vi "Radio Read.vi"() -> ()   [LabVIEW 2013]
uses:
  <vilib>/Instr/_visa.llb/VISA Configure Serial Port (Instr).vi
panel:
  out "Z":dbl(slide) scale=-90.0..90.0
  out "Y":dbl(slide) scale=-90.0..90.0
  out "X":dbl(slide) scale=-90.0..90.0
  out "ELEV":dbl(slide) scale=1000.0..2000.0
  out "ALE":dbl(slide) scale=1000.0..2000.0
  out "THRO":dbl(slide) scale=1000.0..2000.0
  out "RUDD":dbl(slide) scale=1000.0..2000.0
  in  "Stop Button":bool
  out "read buffer":string
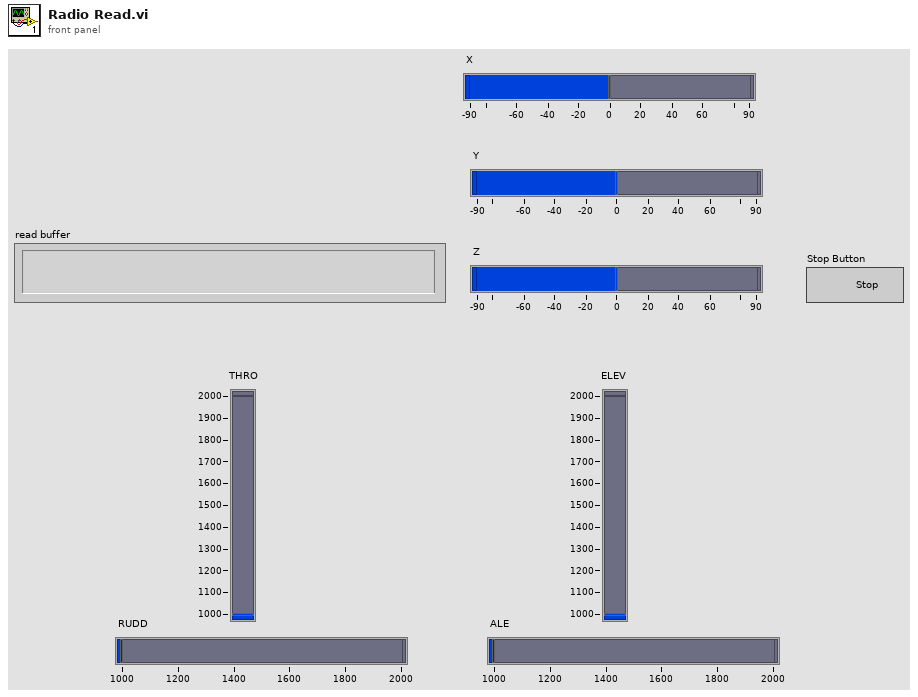
[diagram p1: front panel]
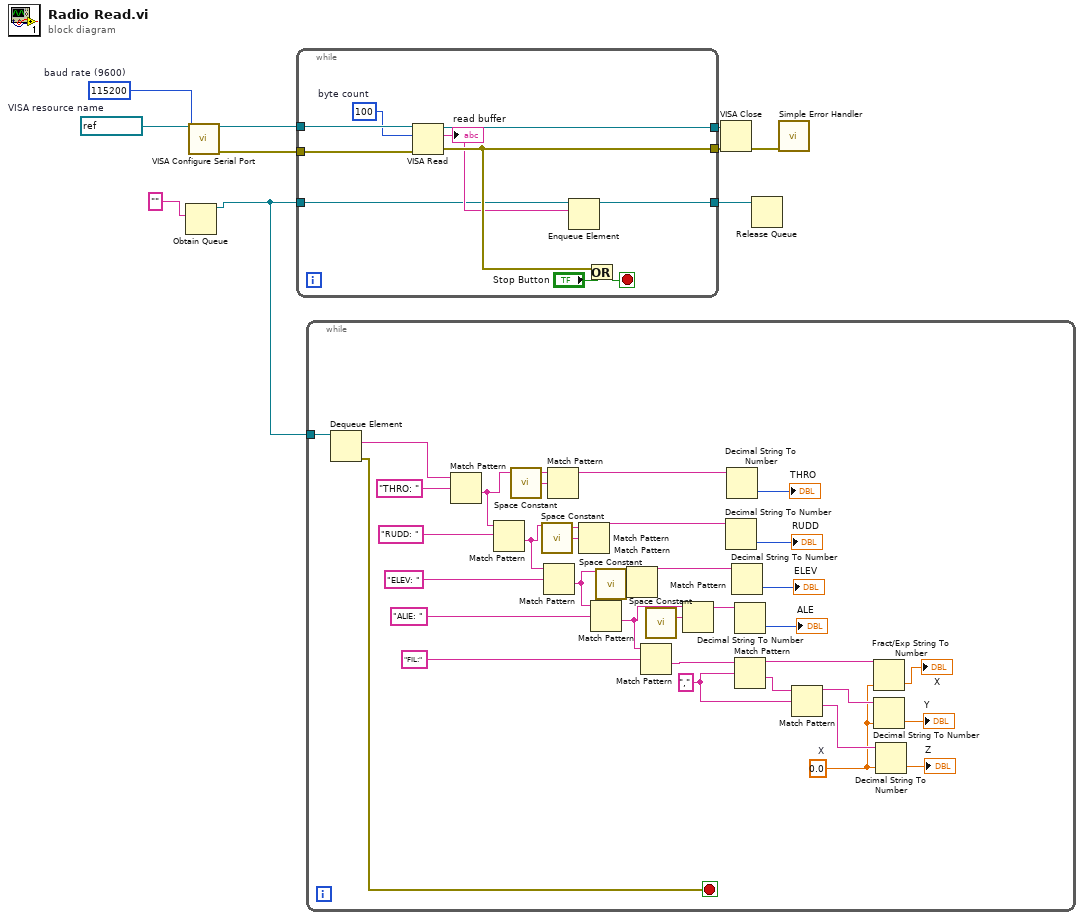
[diagram p0: block diagram]
diagram:
  w1 = u32 115200  # baud rate (9600)
  w8 = refnum<visa-resource-name> "COM3"  # VISA resource name
  n1 = Obtain Queue(element data type="") -> (queue out=w3:refnum<queue>)  [unwired: 4 in, 2 out]
  n2 = call-poly "VISA Configure Serial Port"("VISA resource name"=w8, "baud rate (9600)"=w1) -> ("VISA resource name out"=w6:refnum<visa-resource-name>, "error out"=w7:errorcluster)  [unwired: 12 in]
  n3 = while {
    tunnel: [w20] -> w10
    tunnel: [w18] -> w9
    tunnel: w7 -> [w19]
    tunnel: w6 -> [w15]
    tunnel: w3 -> [w12]
    tunnel: [w11] -> w2
    stop <- w16 stop-if-true
    w14 = u32 100  # byte count
    n4 = VISA Read(VISA resource name=w15, byte count=w14, error in (no error)=w19) -> (VISA resource name out=w20:refnum<visa-resource-name>, read buffer=w13:string, error out=w18:errorcluster)  [unwired: 1 out]
    "read buffer" <- w13
    n5 = Enqueue Element(queue=w12, element=w13) -> (queue out=w11:refnum<queue>)  [unwired: 2 in, 2 out]
    n6 = Or(x=w18, y="Stop Button") -> (x .or. y?=w16:bool)
  }
  n7 = while {
    tunnel: w3 -> [w54]
    stop <- w48 stop-if-true
    w22 = 0.0  # X
    w28 = "," ("regular expression")
    n8 = Dequeue Element(queue=w54) -> (element=w52:string, error out=w48:errorcluster)  [unwired: 2 in, 2 out]
    n9 = Match Pattern(string=w52, regular expression="THRO: ") -> (after substring=w49:string)  [unwired: 1 in, 3 out]
    n10 = Match Pattern(string=w49, regular expression="RUDD: ") -> (after substring=w44:string)  [unwired: 1 in, 3 out]
    n11 = call <vilib>:"Space Constant.vi"() -> ("String"=w51:string)
    n12 = call <vilib>:"Space Constant.vi"() -> ("String"=w50:string)
    n13 = Match Pattern(string=w44, regular expression="ELEV: ") -> (after substring=w33:string)  [unwired: 1 in, 3 out]
    n14 = Match Pattern(string=w49, regular expression=w51) -> (before substring=w38:string)  [unwired: 1 in, 3 out]
    n15 = Match Pattern(string=w44, regular expression=w50) -> (before substring=w39:string)  [unwired: 1 in, 3 out]
    n16 = Match Pattern(string=w33, regular expression="ALIE: ") -> (after substring=w32:string)  [unwired: 1 in, 3 out]
    n17 = call <vilib>:"Space Constant.vi"() -> ("String"=w43:string)
    n18 = Match Pattern(string=w33, regular expression=w43) -> (before substring=w40:string)  [unwired: 1 in, 3 out]
    n19 = Match Pattern(string=w32, regular expression="FIL:") -> (after substring=w30:string)  [unwired: 1 in, 3 out]
    n20 = call <vilib>:"Space Constant.vi"() -> ("String"=w42:string)
    n21 = Match Pattern(string=w32, regular expression=w42) -> (before substring=w41:string)  [unwired: 1 in, 3 out]
    n22 = Decimal String To Number(string=w39) -> (number=→"RUDD":i32)  [unwired: 2 in, 1 out]
    n23 = Decimal String To Number(string=w38) -> (number=→"THRO":i32)  [unwired: 2 in, 1 out]
    n24 = Decimal String To Number(string=w40) -> (number=→"ELEV":i32)  [unwired: 2 in, 1 out]
    n25 = Decimal String To Number(string=w41) -> (number=→"ALE":i32)  [unwired: 2 in, 1 out]
    n26 = Match Pattern(string=w30, regular expression=w28) -> (before substring=w27:string, after substring=w29:string)  [unwired: 1 in, 2 out]
    n27 = Match Pattern(string=w29, regular expression=w28) -> (before substring=w26:string, after substring=w25:string)  [unwired: 1 in, 2 out]
    n28 = Fract/Exp String To Number(string=w27, default (0 dbl)=w22) -> (number=→"X":dbl)  [unwired: 2 in, 1 out]
    n29 = Decimal String To Number(string=w26, default (0L)=w22) -> (number=→"Y":dbl)  [unwired: 1 in, 1 out]
    n30 = Decimal String To Number(string=w25, default (0L)=w22) -> (number=→"Z":dbl)  [unwired: 1 in, 1 out]
  }
  n31 = VISA Close(VISA resource name=w10, error in (no error)=w9) -> (error out=w5:errorcluster)
  n32 = Release Queue(queue=w2) -> ()  [unwired: 2 in, 3 out]
  n33 = call <vilib>:"Simple Error Handler.vi"("error in (no error)"=w5) -> ()  [unwired: 4 in, 5 out]
